vi "Filte Data.vi"(8 "error in (no error)":errorcluster caption="错误输入（无错误）", 11 "Data Viewer 输入":refnum<class "Data Viewer.lvclass">) -> (0 "error out":errorcluster caption="错误输出", 3 "Data Viewer 输出":refnum<class "Data Viewer.lvclass">)   [LabVIEW 2020, in "Data Viewer.lvlib" / "Data Viewer.lvclass"]
uses:
  Data Viewer.lvclass
  <vilib>/Analysis/NI_AALBase.lvlib
  <vilib>/Analysis/3filter.llb/Filter Passband Type.ctl
  <vilib>/Analysis/3filter.llb/Butterworth Filter (DBL).vi
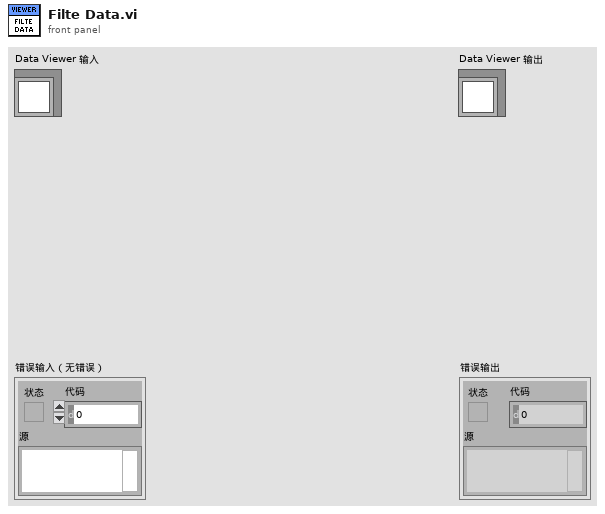
[diagram p1: front panel]
types:
  T1 = typedef "NI_AALBase.lvlib/Filter Passband Type.ctl" = enum32{"Lowpass", "Highpass", "Bandpass", "Bandstop"}
  T2 = typedef "Data Viewer.lvlib/Data Serie--cluster.ctl" = cluster{"Name":string, "Unit":string, "Sample Rate[Hz]":dbl, "Delta t[S]":dbl, "t0":timestamp, "Length":i32, "Time":timestamp[], "Value":dbl[]}
  T3 = typedef "DataSave.lvlib/Data Viewer.lvlib/Data Viewer.lvclass/Filter Type.ctl" = enum16{"Butterworth滤波器", "中值滤波器"}
  T4 = typedef "Filte Method.ctl" = enum16{"低通", "高通", "带通", "带阻"}
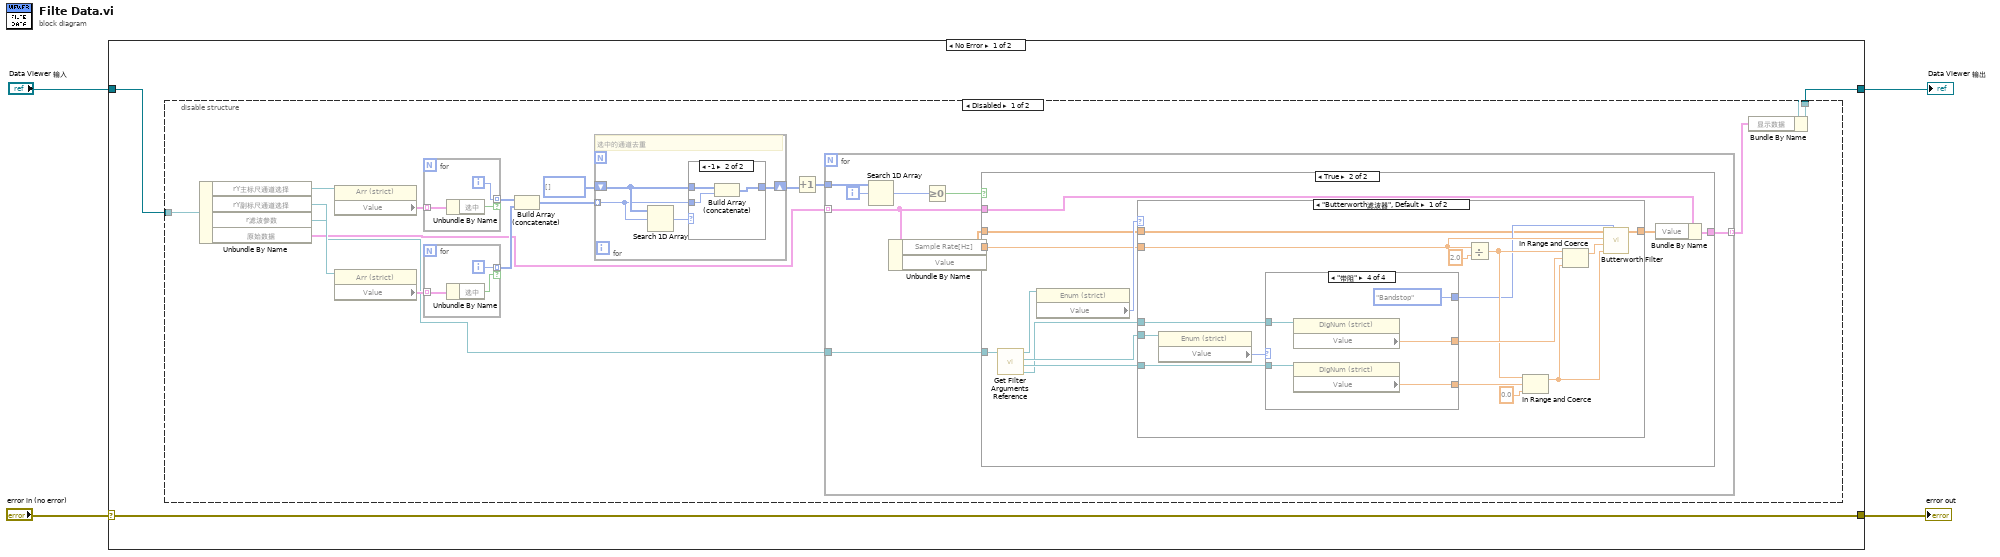
[diagram p0: block diagram]
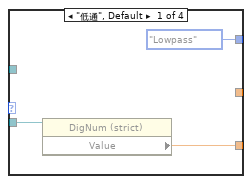
[diagram p3: hidden frame]
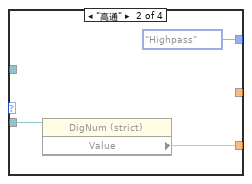
[diagram p4: hidden frame]
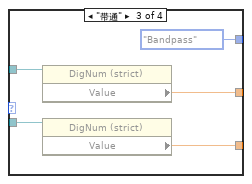
[diagram p5: hidden frame]
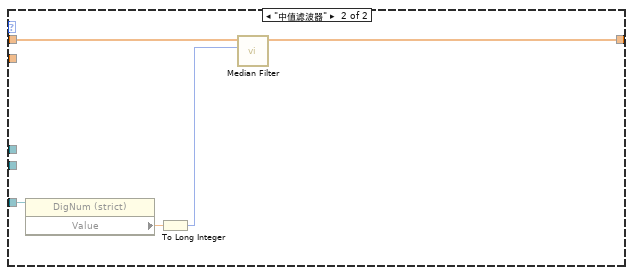
[diagram p6: hidden frame]
diagram:
  n1 = case shown="No Error" "error in (no error)" {
    selector: "error in (no error)" -> [w7 w95]
    tunnel: [w7 w95] -> w3
    tunnel: [w5 w94] -> w1
    tunnel: "Data Viewer 输入" -> [w6 w94]
    frame No Error {
      n2 = disable-structure shown="Disabled" {
        disable-tunnel: w6 -> [w22 _]
        disable-tunnel: [w9 _] -> w5
        frame Disabled {
          n3 = Unbundle By Name(w22) -> ("rY主标尺通道选择"=w19:refnum<vi>, "rY副标尺通道选择"=w18:refnum<vi>, "r滤波参数"=w10:refnum<vi>, "原始数据"=w12:T2[])
          n4 = property class="Arr (strict)"(reference=w19) -> ("Value"=w20:cluster{"选中":bool, "名称":string}[])  [unwired: 1 in, 2 out]
          n5 = property class="Arr (strict)"(reference=w18) -> ("Value"=w21:cluster{"选中":bool, "名称":string}[])  [unwired: 1 in, 2 out]
          n6 = for {
            tunnel: w20 -> [w90] mode=indexing
            tunnel: [w88] -> w17 mode=indexing if=w89
            i -> [w88]
            n7 = Unbundle By Name(w90) -> ("选中"=w89:bool)
          }
          n8 = for {
            tunnel: w21 -> [w93] mode=indexing
            tunnel: [w91] -> w16 mode=indexing if=w92
            i -> [w91]
            n9 = Unbundle By Name(w93) -> ("选中"=w92:bool)
          }
          n10 = Build Array (concatenate)(w17, w16) -> (w14:i32[])
          n11 = for {
            tunnel: w14 -> [w81] mode=indexing
            shift-right: [w80] -> w13
            shift-left: i32[] [] -> [w83]
            # "选中的通道去重"
            n12 = Search 1D Array(1D array=w83, element=w81) -> (index of element=w82:i32)  [unwired: 1 in]
            n13 = case shown="-1" w82 {
              tunnel: w83 -> [w84 w87]
              tunnel: w81 -> [_ w86]
              tunnel: [w84 w85] -> w80
              frame 0, Default {
              }
              frame -1 {
                n14 = Build Array (concatenate)(w87, w86) -> (w85:i32[])
              }
            }
          }
          n15 = Increment(x=w13) -> (x+1=w11:i32[])
          n16 = for {
            tunnel: w12 -> [w23] mode=indexing
            tunnel: w11 -> [w31]
            tunnel: [w24] -> w8 mode=indexing
            tunnel: w10 -> [w27]
            i -> [w30]
            n17 = Search 1D Array(1D array=w31, element=w30) -> (index of element=w29:i32)  [unwired: 1 in]
            n18 = Unbundle By Name(w23) -> ("Sample Rate[Hz]"=w25:dbl, "Value"=w26:dbl[])
            n19 = Greater Or Equal To 0?(x=w29) -> (x >= 0?=w28:bool)
            n20 = case shown="True" w28 {
              tunnel: w27 -> [_ w43]
              tunnel: w26 -> [_ w39]
              tunnel: w25 -> [_ w38]
              tunnel: [w32 w36] -> w24
              tunnel: w23 -> [w32 w35]
              frame False {
              }
              frame True {
                n21 = call "Get Filter Arguments Reference.vi"("滤波参数引用"=w43) -> ("参数2"=w33:refnum<vi>, "参数1"=w34:refnum<vi>, "滤波方式"=w40:refnum<vi>, "滤波器类型"=w42:refnum<vi>)  [unwired: 7 in]
                n22 = property class="Enum (strict)"(reference=w42) -> ("Value"=w41:T3)  [unwired: 1 in, 2 out]
                n23 = case shown="\"Butterworth滤波器\", Default" w41 {
                  tunnel: w40 -> [w58 _]
                  tunnel: w39 -> [w45 w79]
                  tunnel: w38 -> [w49 _]
                  tunnel: [w44 w75] -> w37
                  tunnel: w34 -> [w56 w78]
                  tunnel: w33 -> [w55 _]
                  frame "Butterworth滤波器", Default {
                    n24 = property class="Enum (strict)"(reference=w58) -> ("Value"=w57:T4)  [unwired: 1 in, 2 out]
                    n25 = case shown="\"带阻\"" w57 {
                      tunnel: w56 -> [w61 w63 w68 w73]
                      tunnel: [w60 w62 w67 w72] -> w52
                      tunnel: [Filter_Passband_Type."Lowpass" ("filter type") Filter_Passband_Type."Highpass" ("filter type") Filter_Passband_Type."Bandpass" ("filter type") Filter_Passband_Type."Bandstop" ("filter type")] -> w46
                      tunnel: w55 -> [_ _ w66 w71]
                      tunnel: [_ _ w65 w70] -> w51
                      frame "低通", Default {
                        n26 = property class="DigNum (strict)"(reference=w61) -> ("Value"=w60:dbl)  [unwired: 1 in, 2 out]
                      }
                      frame "高通" {
                        n27 = property class="DigNum (strict)"(reference=w63) -> ("Value"=w62:dbl)  [unwired: 1 in, 2 out]
                      }
                      frame "带通" {
                        n28 = property class="DigNum (strict)"(reference=w66) -> ("Value"=w65:dbl)  [unwired: 1 in, 2 out]
                        n29 = property class="DigNum (strict)"(reference=w68) -> ("Value"=w67:dbl)  [unwired: 1 in, 2 out]
                      }
                      frame "带阻" {
                        n30 = property class="DigNum (strict)"(reference=w71) -> ("Value"=w70:dbl)  [unwired: 1 in, 2 out]
                        n31 = property class="DigNum (strict)"(reference=w73) -> ("Value"=w72:dbl)  [unwired: 1 in, 2 out]
                      }
                    }
                    n32 = Divide(x=w49, y=2.0) -> (x/y=w50:dbl)
                    n33 = In Range and Coerce(upper limit=w50, x=w52, lower limit=0.0 ("下限")) -> (coerced(x)=w48:dbl)  [unwired: 1 out]
                    n34 = In Range and Coerce(upper limit=w50, x=w51, lower limit=w48) -> (coerced(x)=w47:dbl)  [unwired: 1 out]
                    n35 = call-poly <vilib>:"Butterworth Filter.vi"("filter type"=w46, "low cutoff freq: fl"=w48, "high cutoff freq: fh"=w47, "sampling freq: fs"=w49, "X"=w45) -> ("Filtered X"=w44:dbl[])  [unwired: 3 in, 1 out]
                  }
                  frame "中值滤波器" {
                    n36 = property class="DigNum (strict)"(reference=w78) -> ("Value"=w77:dbl)  [unwired: 1 in, 2 out]
                    n37 = To Long Integer(number=w77) -> (32bit integer=w76:i32)
                    n38 = call <vilib>:"Median Filter.vi"("left rank"=w76, "X"=w79) -> ("Filtered X"=w75:dbl[])  [unwired: 8 in, 1 out]
                  }
                }
                n39 = Bundle By Name(cluster=w35, "Value"=w37) -> (w36:T2)
              }
            }
          }
          n40 = Bundle By Name(cluster=w22, "显示数据"=w8) -> (w9:refnum<class "Data Viewer.lvclass">)
        }
        frame Enabled {
        }
      }
    }
    frame Error {
    }
  }
  "error out" <- w3
  "Data Viewer 输出" <- w1
